vi "TrigTest.vi"() -> ()   [LabVIEW 2021]
uses:
  <vilib>/DAQmx/read.llb/DAQmx Read (Analog 1D Wfm NChan NSamp).vi
  <vilib>/DAQmx/create/channels.llb/DAQmx Create Channel (AI-Acceleration-Accelerometer).vi
  <vilib>/DAQmx/configure/timing.llb/DAQmx Timing (Sample Clock).vi
  <vilib>/DAQmx/miscellaneous.llb/DAQmx Fill In Error Info.vi
  <vilib>/express/express analysis/Spectral/Block/exnSpectralBlock spectral measurements PSD poly.vi
  <vilib>/express/express analysis/Spectral/Block/exnSpectralBlock spectral measurements PSD array WFM.vi
  <vilib>/express/express analysis/Spectral/XNode/ExpressSpectralMeasurementsBlockNode.xnode
  <resource>/objmgr/daqmx.rc
panel:
  out "Filename Out":path
  out "Reference Accelerometer On":bool caption="Saving Data"
  out "Saving Data":bool
  in  "Filename":path=path "C:/Users/joud/Dropbox/Satme_2024_IEEE_Edge_Processing_Compensator/Data/Benchtop Test/Frequency Sweep V2/Ref.lvm"
  in  "Enable":bool=TRUE
  out "data 2":cluster{"f0":dbl, "df":dbl, "magnitude":dbl[]}[](graph) caption="PSD"
  out "data":waveform(dbl)[](graph) caption="Ref Acc"
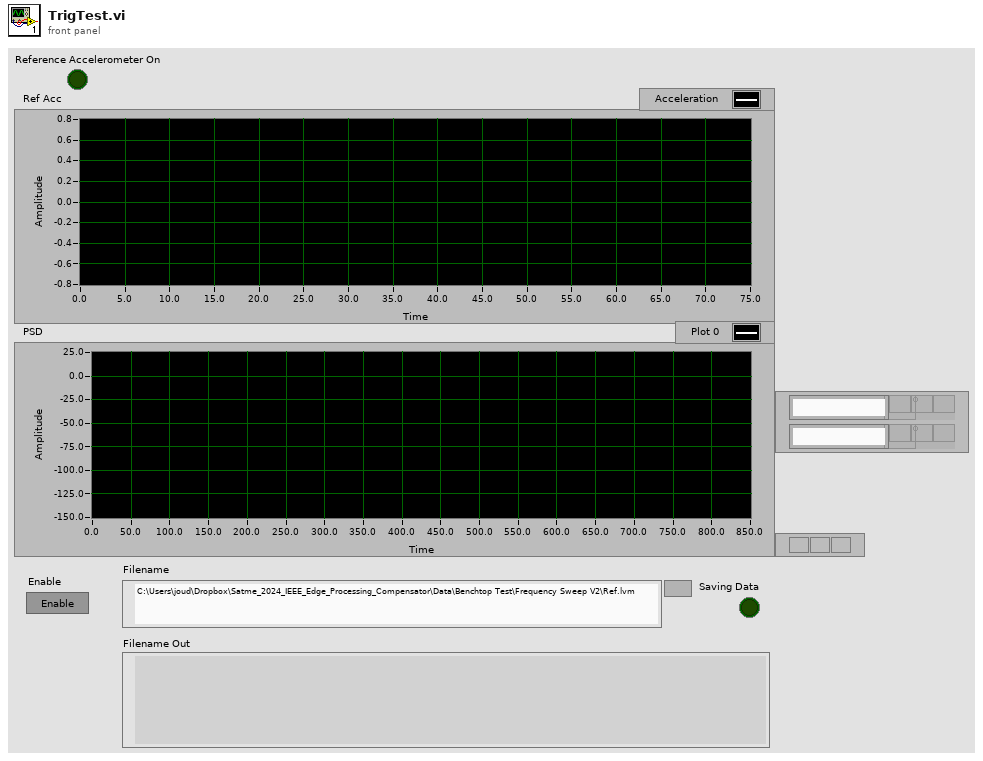
[diagram p1: front panel]
types:
  T1 = cluster{"averaging mode":u16, "weighting mode":u16, "number of averages":u32}
  T2 = cluster{"dB On (F)":bool, "unwrap phase (F)":bool, "convert to degree (F)":bool}
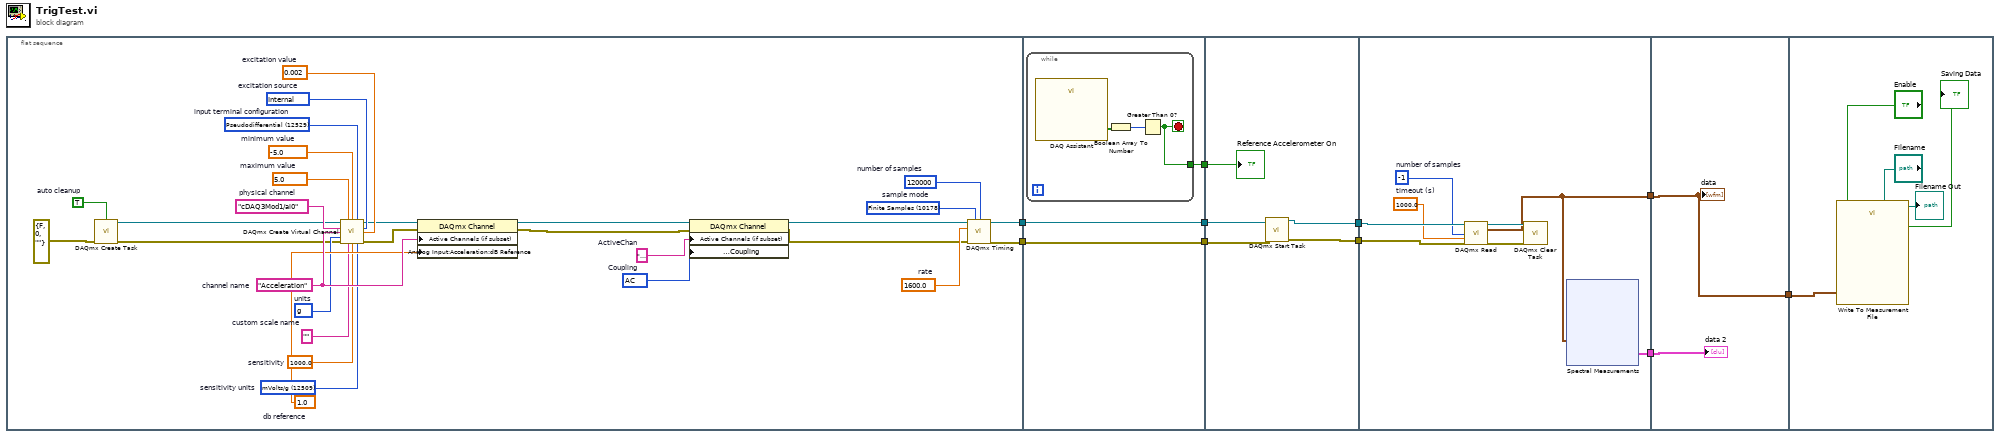
[diagram p0: block diagram]
diagram:
  n1 = flat-sequence {
    tunnel: [w12] -> w10
    tunnel: [w11] -> w9
    tunnel: w10 -> [w42]
    tunnel: w9 -> [w41]
    tunnel: [w42] -> w8
    tunnel: [w41] -> w7
    tunnel: [w40] -> w1
    tunnel: w8 -> [w50]
    tunnel: w7 -> [w49]
    tunnel: [w48] -> w6
    tunnel: [w47] -> w5
    tunnel: w1 -> [w46]
    tunnel: w6 -> [w56]
    tunnel: w5 -> [w53]
    tunnel: [w52] -> w4
    tunnel: [w51] -> w3
    tunnel: w4 -> [w68]
    tunnel: w3 -> [w69]
    tunnel: [w68] -> w2
    tunnel: w2 -> [w74]
    frame #0 {
      w38 = 10178 items=["Finite Samples"=10178, "Continuous Samples"=10123, "Hardware Timed Single Point"=12522]  # sample mode
      w37 = 120000  # number of samples
      w36 = 1600.0  # rate
      w32 = 10045 items=["AC"=10045, "DC"=10050, "GND"=10066]  # Coupling
      w31 = "Acceleration"  # ActiveChan
      w29 = 1.0  # db reference
      w26 = 10186 items=["g"=10186, "m/s^2"=12470, "From Custom Scale"=10065]  # units
      w25 = 12529 items=["default"=-1, "RSE"=10083, "NRSE"=10078, "Differential"=10106, "Pseudodifferential"=12529]  # input terminal configuration
      w24 = 10200 items=["Internal"=10200, "External"=10167, "None"=10230]  # excitation source
      w23 = 0.002  # excitation value
      w22 = 12509 items=["mVolts/g"=12509, "Volts/g"=12510]  # sensitivity units
      w21 = 1000.0  # sensitivity
      w30 = "Acceleration"  # channel name
      w19 = ""  # custom scale name
      w18 = -5.0  # minimum value
      w17 = 5.0  # maximum value
      w16 = "cDAQ3Mod1/ai0"  # physical channel
      w14 = TRUE  # auto cleanup
      n2 = call <vilib>:"DAQmx Create Task.vi"("auto cleanup"=w14, "error in"=errorcluster {"status"=FALSE, "code"=0, "source"=""}) -> ("task out"=w15:refnum<k21>, "error out"=w13:errorcluster)  [unwired: 12 in]
      n3 = call-poly <vilib>:"DAQmx Create Virtual Channel.vi"("task in"=w15, "maximum value"=w17, "minimum value"=w18, "input terminal configuration"=w25, "physical channels"=w16, "current excitation source"=w24, "name to assign"=w30, "current excitation value"=w23, "units"=w26, "error in"=w13, "custom scale name"=w19, "sensitivity"=w21, "sensitivity units"=w22) -> ("task out"=w20:refnum<k21>, "error out"=w27:errorcluster)  [unwired: 1 in]
      n4 = property class="DAQmx Channel"(reference=w20, error in=w27, "Active Channels (if subset)"=w30, "Analog Input:Acceleration:dB Reference"=w29) -> (reference out=w34:refnum<k21>, error out=w28:errorcluster)
      n5 = property class="DAQmx Channel"(reference=w34, error in=w28, "Active Channels (if subset)"=w31, "Analog Input:General Properties:Input Configuration:Coupling"=w32) -> (reference out=w35:refnum<k21>, error out=w33:errorcluster)
      n6 = call-poly <vilib>:"DAQmx Timing.vi"("task/channels in"=w35, "sample mode"=w38, "samples per channel"=w37, "rate"=w36, "error in"=w33) -> ("task out"=w12:refnum<k21>, "error out"=w11:errorcluster)  [unwired: 9 in]
    }
    frame #1 {
      n7 = while {
        tunnel: [w43] -> w40
        stop <- w43 stop-if-true
        n8 = call "DAQ Assistant"() -> ("data"=w45:bool[])  [unwired: 17 in, 2 out]
        n9 = Boolean Array To Number(Boolean array=w45) -> (number=w44:u32)
        n10 = Greater Than 0?(x=w44) -> (x > 0?=w43:bool)
      }
    }
    frame #2 {
      n11 = call <vilib>:"DAQmx Start Task.vi"("task/channels in"=w50, "error in"=w49) -> ("task out"=w48:refnum<k21>, "error out"=w47:errorcluster)  [unwired: 12 in]
      "Reference Accelerometer On" <- w46
    }
    frame #3 {
      w54 = 1000.0  # timeout (s)
      w55 = -1  # number of samples
      n12 = call-poly <vilib>:"DAQmx Read.vi"("task/channels in"=w56, "number of samples per channel"=w55, "timeout"=w54, "error in"=w53) -> ("task out"=w58:refnum<k21>, "data"=w52:waveform(dbl)[], "error out"=w57:errorcluster)  [unwired: 9 in]
      n13 = call <vilib>:"DAQmx Clear Task.vi"("task in"=w58, "error in"=w57) -> ()  [unwired: 13 in, 1 out]
      n14 = xnode "Spectral Measurements"("Signals"=w52) -> ("PSD"=w51:cluster{"f0":dbl, "df":dbl, "magnitude":dbl[]}[])  [unwired: 1 in, 1 out]
    }
    frame #4 {
      "data" <- w68
      "data 2" <- w69
    }
    frame #5 {
      n15 = call "Write To Measurement File"("Signals"=w74, "Enable"="Enable", "Filename"="Filename") -> ("Filename Out"=→"Filename Out":path, "Saving Data"=→"Saving Data":bool)  [unwired: 14 in, 1 out]
    }
  }
